vi "Inspector Template [VarMan Spy].vi"() -> ()   [LabVIEW 2021]
doc: "::: CalcExpress Toolkit :::\nCopyright (c) 2000-2026 Konstantin Shifershteyn. All rights reserved."
uses:
  vi.lib/addons/CalcExpress/cetypes.llb/VarMan Variable Context Handle.ctl
  vi.lib/addons/CalcExpress/cemisc.llb/[ce] CE component paths - Kind of Path Enum.ctl
  <vilib>/Utility/miscctls.llb/LVBoundsTypeDef.ctl
panel:
  out "I32B":i32 caption="Bit-keeping conversion" format="%.0x"
  out "I32M":i32 caption="Saturating conversion" format="%.0x"
  out "writerID":u32 caption="writer ID"
  in  "%write":bool
  in  "EnaWrap":bool=TRUE caption="Wrap"
  in  "ShowInt32":bool caption="show I32 and U32"
  out "h_IR":T1(array[cluster]) {"timestamp" format="%<%H:%M:%S%2u\n%d/%m/%Y>T"}
  out "h_any":T2(array[cluster]) {"timestamp" format="%<%H:%M:%S%2u\n%d/%m/%Y>T"}
  out "h_a2str":T3(array[cluster]) {"timestamp" format="%<%H:%M:%S%2u\n%d/%m/%Y>T"}
  out "h_a1str":T4(array[cluster]) {"timestamp" format="%<%H:%M:%S%2u\n%d/%m/%Y>T"}
  out "h_a2cdb":T5(array[cluster]) {"value"."data" format="%.2f"; "timestamp" format="%<%H:%M:%S%2u\n%d/%m/%Y>T"}
  out "h_a1cdb":T6(array[cluster]) {"value"."data" format="%.2f"; "timestamp" format="%<%H:%M:%S%2u\n%d/%m/%Y>T"}
  out "h_cdb":T7(array[cluster]) {"value" format="%.2f"; "timestamp" format="%<%H:%M:%S%2u\n%d/%m/%Y>T"}
  out "h_a2dbl":T8(array[cluster]) {"value"."data" format="%.2f"; "timestamp" format="%<%H:%M:%S%2u\n%d/%m/%Y>T"}
  out "IR":cluster{"Initial index":i32, "Final index":i32} caption="Index Range"
  out "h_a1dbl":T9(array[cluster]) {"value"."data" format="%.2f"; "timestamp" format="%<%H:%M:%S%2u\n%d/%m/%Y>T"}
  in  "bndry":string
  in  "%h_Update":bool caption="update [F2]"
  in  "%h_Auto":bool caption="auto update"
  in  "%h_Reverse":bool=TRUE caption="reversed"
  in  "%h_Show":bool caption="History"
  out "dbl":dbl caption="Value" format="%.2f"
  out "h_str":T2(array[cluster]) caption="Variable History" {"timestamp" format="%<%H:%M:%S%2u\n%d/%m/%Y>T"}
  out "h_dbl":T10(array[cluster]) caption="Variable History" {"value" format="%.2f"; "timestamp" format="%<%H:%M:%S%2u\n%d/%m/%Y>T"}
  in  "alias":string
  out "var type":i32(ring)=10 items=["String"=0, "DBL Number"=1, "Identifier"=2, "1D Array of DBL"=3, "2D Array of DBL"=4, "CDB Number"=5, "1D Array of CDB"=6, "2D Array of CDB"=7, "1D Array of String"=8, "2D Array of String"=9, "Unknown data type"=10, "Index Range"=252]
  in  "var name":string
  out "any":string
  out "a2dbl":dbl[][](array[numeric]) format="%.2f"
  out "a2cdb":cdb[][](array[numeric]) format="%.2f"
  out "cdb":cdb caption="Value" format="%.2f"
  out "a1cdb":cdb[](array[numeric]) format="%.2f"
  out "a1dbl":dbl[](array[numeric]) format="%.2f"
  out "a2str":string[][](array[string])
  out "a1str":string[](array[string])
  in  "Display style":u32(ring) caption="Style" items=["Normal", "'\\' Code", "Password", "Hex dump"]
  out "Update TS":dbl=3131888400.0 format="%<%H:%M:%S%1u>T"
  out "str":string
  in  "Precision":u8=2 caption="prec"
  in  "Format":u8(ring) items=["Floating point", "Scientific", "Engineering", "Binary", "Octal", "Hexadecimal", "Relative time", "Absolute time"]
  in  "%Pause":bool
  out "Context":string
  out "Variable":string
  in  "handle":T11=-1
  # ":"
  # ":"
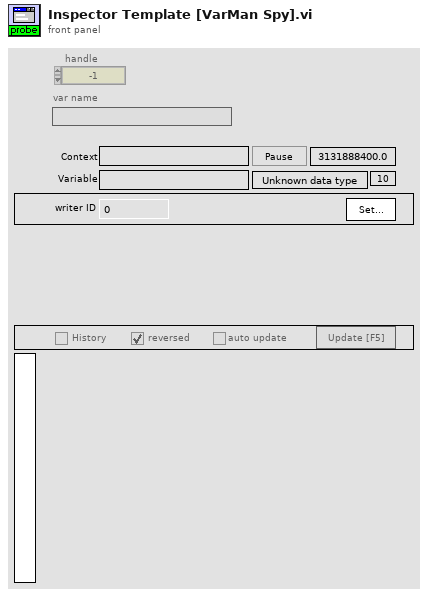
[diagram p1: front panel]
types:
  T1 = cluster{"timestamp":dbl, "IR 2":cluster{"Initial index":i32, "Final index":i32}, "writerID":u32}[]
  T2 = cluster{"timestamp":dbl, "value":string, "writerID":u32}[]
  T3 = cluster{"timestamp":dbl, "value":cluster{"data":string[][]}, "writerID":u32}[]
  T4 = cluster{"timestamp":dbl, "value":cluster{"data":string[]}, "writerID":u32}[]
  T5 = cluster{"timestamp":dbl, "value":cluster{"data":cdb[][]}, "writerID":u32}[]
  T6 = cluster{"timestamp":dbl, "value":cluster{"data":cdb[]}, "writerID":u32}[]
  T7 = cluster{"timestamp":dbl, "value":cdb, "writerID":u32}[]
  T8 = cluster{"timestamp":dbl, "value":cluster{"data":dbl[][]}, "writerID":u32}[]
  T9 = cluster{"timestamp":dbl, "value":cluster{"data":dbl[]}, "writerID":u32}[]
  T10 = cluster{"timestamp":dbl, "value":dbl, "writerID":u32}[]
  T11 = typedef "VarMan Variable Context Handle.ctl" = i32
  T12 = typedef "LVBoundsTypeDef.ctl" = cluster{"Width":u32, "Height":u32}
  T13 = typedef "LVPositionTypeDef.ctl" = cluster{"Left":i32, "Top":i32}
  T14 = typedef "VarMan Variable Data Statistics.ctl" = cluster{"writer ID":u32, "write MS":u32, "write TS":dbl, "write Cnt":u32}
  T15 = cluster{"timestamp":dbl, "value":string, "value":u32}[]
  T16 = cluster{"timestamp":dbl, "value":dbl, "value":u32}[]
  T17 = cluster{"timestamp":dbl, "value":cluster{"data":dbl[]}, "value":u32}[]
  T18 = cluster{"timestamp":dbl, "value":cluster{"data":dbl[][]}, "value":u32}[]
  T19 = cluster{"timestamp":dbl, "value":cdb, "value":u32}[]
  T20 = cluster{"timestamp":dbl, "value":cluster{"data":cdb[]}, "value":u32}[]
  T21 = cluster{"timestamp":dbl, "value":cluster{"data":cdb[][]}, "value":u32}[]
  T22 = cluster{"timestamp":dbl, "value":cluster{"data":string[]}, "value":u32}[]
  T23 = cluster{"timestamp":dbl, "value":cluster{"data":string[][]}, "value":u32}[]
  T24 = cluster{"timestamp":dbl, "Index Range":cluster{"Initial index":i32, "Final index":i32}, "value":u32}[]
  T25 = enum32{"invalid app kind", "Development System", "Run Time System", "Student Edition", "Embedded LabVIEW", "Evaluation", "Custom"}
  T26 = typedef "[ce] CE component paths - Kind of Path Enum.ctl" = enum16{"VIs", "FuncVIs", "Help", "Examples", "Project", "Templates"}
  T27 = enum32{"Invalid", "Standard", "Closed", "Hidden", "Minimized", "Maximized"}
  T28 = typedef "eventvkey.ctl" = enum16{"ASCII", "Enter", "Return", "Shift", "Ctrl", "Alt", "Cmd", "Opt", "Caps", "NumLock", "Clear", "Break", "Up", "Down", "Left", "Right", "Insert", "Delete", "Home", "End", "PageUp", "PageDown", "Escape", "Help", "Pause", "ScrollLock", "F1", "F2", "F3", "F4", "F5", "F6", "F7", "F8", "F9", "F10", "F11", "F12", "F13", "F14", "F15", "F16", "F17", "F18", "F19", "F20", "F21", "F22", "F23", "F24", "Play", "VolumeUp", "VolumeDown", "Mute", "Two Byte Char"}
  T29 = cluster{"Shift":bool, "Ctrl":bool, "Alt":bool, "Cmd":bool, "Opt":bool}
  T30 = typedef "LVRectTypeDef.ctl" = cluster{"Left":i16, "Top":i16, "Right":i16, "Bottom":i16}
  T31 = cluster{"Left":i32, "Top":i32, "Right":i32, "Bottom":i32}
  T32 = cluster{"Value":u8, "Value":u8, "Value":bool, "Value":u32, "Value":bool}
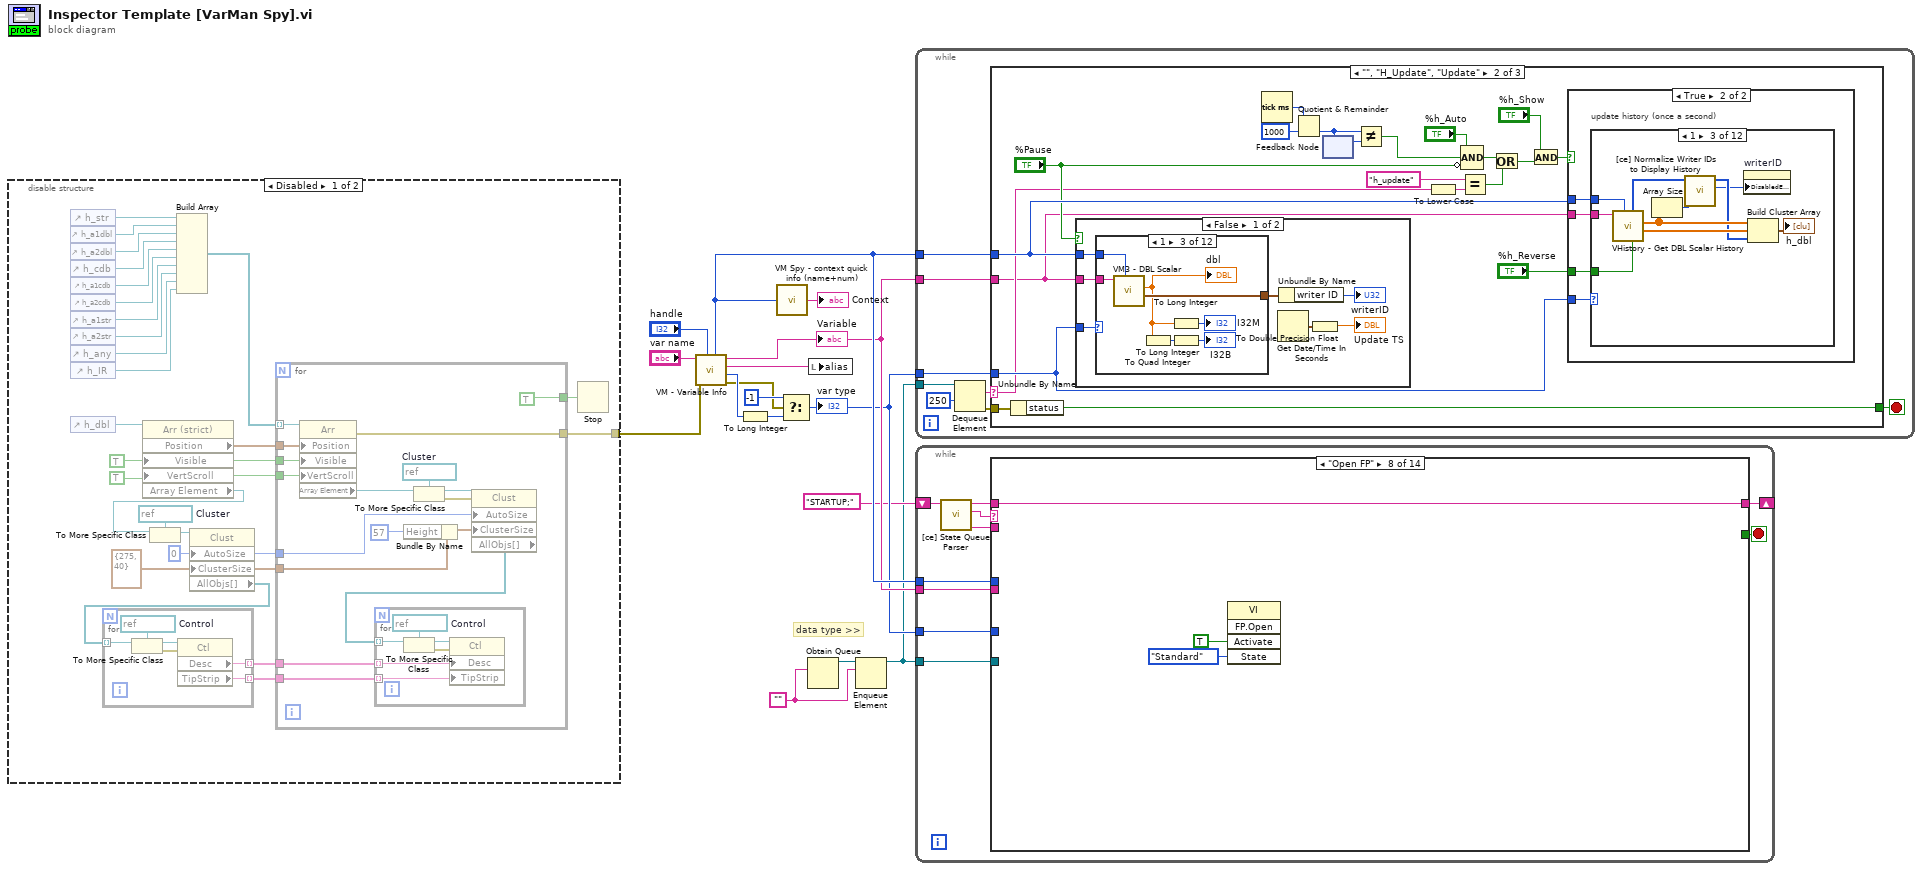
[diagram p0: block diagram]
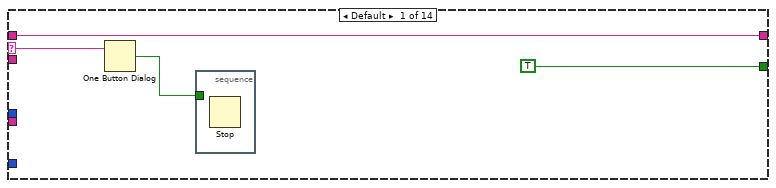
[diagram p3: hidden frame]
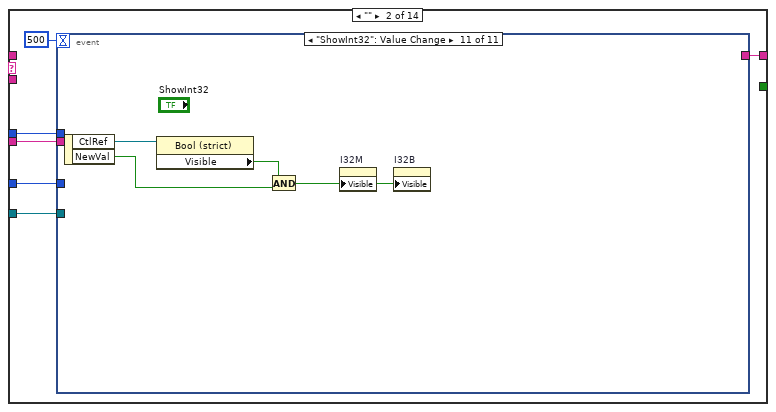
[diagram p4: hidden frame]
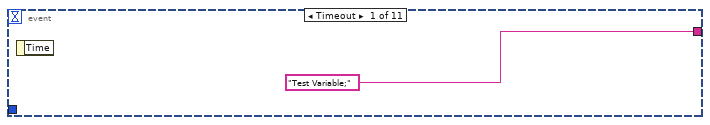
[diagram p5: hidden frame]
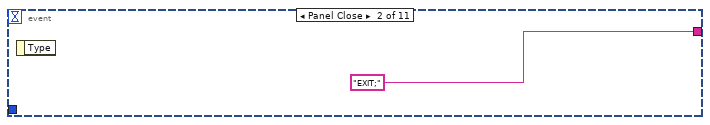
[diagram p6: hidden frame]
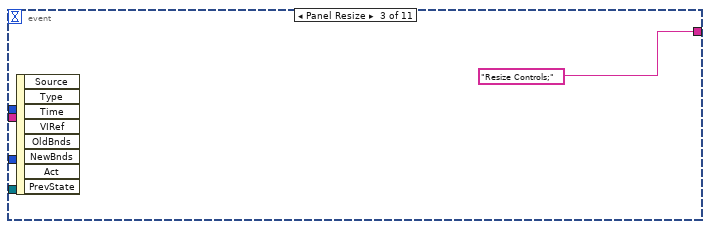
[diagram p7: hidden frame]
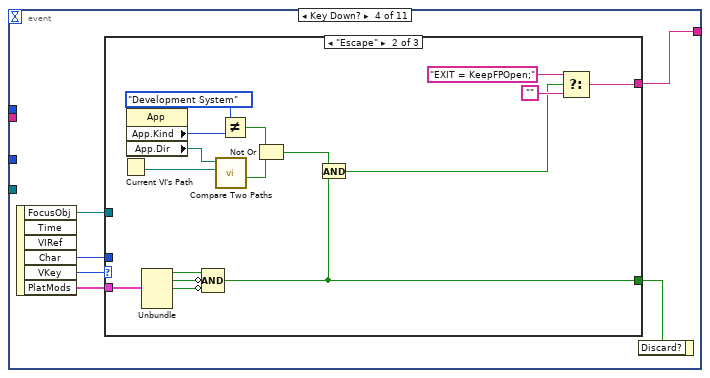
[diagram p8: hidden frame]
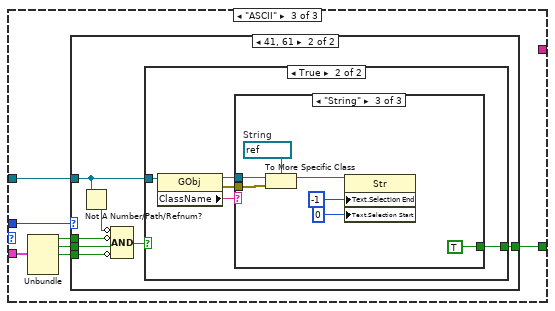
[diagram p10: hidden frame]
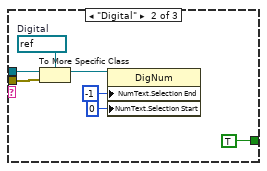
[diagram p14: hidden frame]
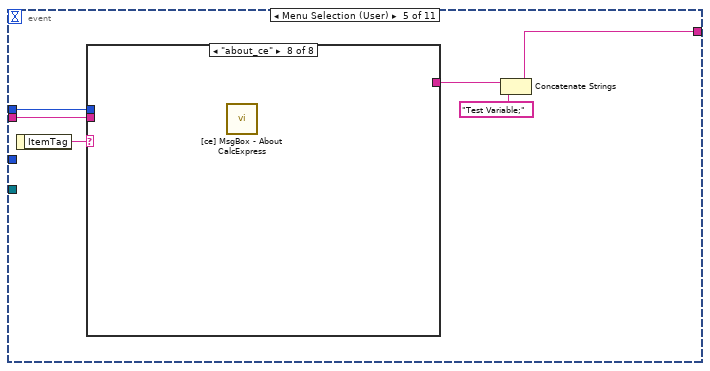
[diagram p15: hidden frame]
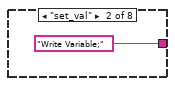
[diagram p17: hidden frame]
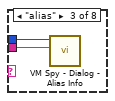
[diagram p18: hidden frame]
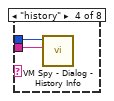
[diagram p19: hidden frame]
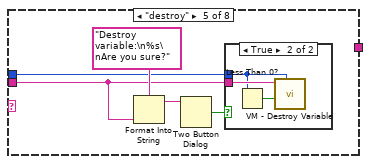
[diagram p20: hidden frame]
diagram:
  w2 = ""
  # "data type >>"
  n1 = disable-structure shown="Disabled" {
    disable-tunnel: [w19 _] -> w1
    frame Disabled {
      w17 = TRUE
      w31 = TRUE ("Visible")
      w27 = T12 {"Width"=275, "Height"=40} ("Cluster Size")
      w26 = u32 0 ("Auto Sizing")
      w23 = refnum<vi> refnum  # Cluster
      n2 = control-ref of="h_str"() -> (w41:refnum<vi>)
      n3 = control-ref of="h_a1dbl"() -> (w40:refnum<vi>)
      n4 = control-ref of="h_a2dbl"() -> (w39:refnum<vi>)
      n5 = control-ref of="h_cdb"() -> (w38:refnum<vi>)
      n6 = control-ref of="h_a1cdb"() -> (w37:refnum<vi>)
      n7 = control-ref of="h_a2cdb"() -> (w36:refnum<vi>)
      n8 = control-ref of="h_a1str"() -> (w35:refnum<vi>)
      n9 = control-ref of="h_a2str"() -> (w34:refnum<vi>)
      n10 = control-ref of="h_any"() -> (w33:refnum<vi>)
      n11 = control-ref of="h_IR"() -> (w32:refnum<vi>)
      n12 = control-ref of="h_dbl"() -> (w21:refnum<vi>)
      n13 = property class="Arr (strict)"(reference=w21, "Visible"=w31, "VertScroll"=w17) -> ("Position"=w22:T13, "Array Element"=w24:refnum<vi>)  [unwired: 1 in, 2 out]
      n14 = To More Specific Class(target class=w23, reference=w24) -> (specific class reference=w25:refnum<vi>)  [unwired: 1 in, 1 out]
      n15 = Build Array(w41, w40, w39, w38, w37, w36, w35, w34, w33, w32) -> (w20:refnum<vi>[])
      n16 = property class="Clust"(reference=w25, "AutoSize"=w26, "ClusterSize"=w27) -> ("AllObjs[]"=w28:refnum<vi>[])  [unwired: 1 in, 2 out]
      n17 = for {
        tunnel: w28 -> [w46] mode=indexing
        tunnel: [w43] -> w29 mode=indexing
        tunnel: [w42] -> w30 mode=indexing
        w47 = refnum<vi> refnum  # Control
        n18 = To More Specific Class(target class=w47, reference=w46) -> (specific class reference=w45:refnum<vi>, error out=w44:errorcluster)  [unwired: 1 in]
        n19 = property class="Ctl"(reference=w45, error in=w44) -> ("Desc"=w43:string, "TipStrip"=w42:string)  [unwired: 2 out]
      }
      n20 = for {
        tunnel: w22 -> [w64]
        tunnel: w20 -> [w63] mode=indexing
        tunnel: w26 -> [w58]
        tunnel: w27 -> [w57]
        tunnel: w29 -> [w53]
        tunnel: w30 -> [w52]
        tunnel: w31 -> [w51]
        tunnel: [w50] -> w19
        tunnel: [TRUE] -> w18
        tunnel: w17 -> [w48]
        w62 = refnum<vi> refnum  # Cluster
        n21 = property class="Arr"(reference=w63, "Position"=w64, "Visible"=w51, "VertScroll"=w48) -> (error out=w50:errorcluster, "Array Element"=w61:refnum<vi>)  [unwired: 1 in, 1 out]
        n22 = Bundle By Name(cluster=w57, "Height"=u32 57) -> (w56:T12)
        n23 = To More Specific Class(target class=w62, reference=w61) -> (specific class reference=w60:refnum<vi>, error out=w59:errorcluster)  [unwired: 1 in]
        n24 = property class="Clust"(reference=w60, error in=w59, "AutoSize"=w58, "ClusterSize"=w56) -> ("AllObjs[]"=w54:refnum<vi>[])  [unwired: 2 out]
        n25 = for {
          tunnel: w54 -> [w69] mode=indexing
          tunnel: w53 -> [w66] mode=indexing
          tunnel: w52 -> [w65] mode=indexing
          w70 = refnum<vi> refnum  # Control
          n26 = To More Specific Class(target class=w70, reference=w69) -> (specific class reference=w68:refnum<vi>, error out=w67:errorcluster)  [unwired: 1 in]
          n27 = property class="Ctl"(reference=w68, error in=w67, "Desc"=w66, "TipStrip"=w65) -> ()  [unwired: 2 out]
        }
      }
      n28 = Stop(stop? (T)=w18) -> ()
    }
    frame Enabled {
    }
  }
  n29 = call "VM - Variable Info.vi"("VC Handle"="handle", "error in"=w1, "name_spec"="var name") -> ("error out"=w5:errorcluster, "var type"=w10:u32, "alias"=w13:string, "var name"=w8:string, "var VC Handle"=w9:T11)  [unwired: 3 in, 1 out]
  "Variable" <- w8
  n30 = To Long Integer(number=w10) -> (32bit integer=w12:i32)
  n31 = call "VM Spy - context quick info (name+num).vi"("handle"=w9) -> ("context info"=→"Context":string)  [unwired: 4 in]
  n32 = Select(t=-1, s=w5, f=w12) -> (s? t:f=w7:i32)
  "var type" <- w7
  n33 = Obtain Queue(element data type=w2) -> (queue out=w4:refnum<queue>)  [unwired: 4 in, 2 out]
  n34 = local write "alias"(w13) -> ()
  n35 = Enqueue Element(queue=w4, element=w2) -> (queue out=w3:refnum<queue>)  [unwired: 2 in, 2 out]
  n36 = while {
    tunnel: w8 -> [w78]
    tunnel: w9 -> [w76]
    tunnel: w7 -> [w77]
    tunnel: w3 -> [w75]
    stop <- w72 stop-if-true
    n37 = Dequeue Element(queue=w75, timeout in ms (-1)=250) -> (element=w74:string, error out=w71:errorcluster)  [unwired: 1 in, 2 out]
    n38 = case shown="\"\", \"H_Update\", \"Update\"" w74 {
      selector: w74 -> [_ w84 _]
      tunnel: w78 -> [_ w80 _]
      tunnel: w77 -> [_ w100 _]
      tunnel: w76 -> [_ w99 _]
      tunnel: [TRUE w86 w278] -> w72
      tunnel: w71 -> [_ w87 w279]
      frame "EXIT" {
      }
      frame "", "H_Update", "Update" {
        n39 = Unbundle By Name(w87) -> ("status"=w86:bool)
        n40 = case shown="False" "%Pause" {
          tunnel: w99 -> [w224 _]
          tunnel: w80 -> [w222 _]
          tunnel: w100 -> [w221 _]
          frame False {
            n41 = case shown="1" w221 {
              selector: w221 -> [_ _ _ _ _ _ _ _ _ _ w270 w276]
              tunnel: w222 -> [w227 w231 w238 w242 w246 w250 w254 w258 w262 w266 w271 w277]
              tunnel: w224 -> [w226 w229 w237 w240 w244 w248 w252 w256 w260 w264 w268 w273]
              tunnel: [w225 w228 w236 w239 w243 w247 w251 w255 w259 w263 w267 w272] -> w219
              frame -1, 2 {
                n42 = call "VM3 - Variable Data Info.vi"("VC Handle"=w226, "name_spec"=w227) -> ("stats"=w225:T14)  [unwired: 4 in, 5 out]
              }
              frame 0 {
                n43 = call "VM3 - String.vi"("VC Handle"=w229, "name_spec"=w231) -> ("stats"=w228:T14, "value out"=→"str":string)  [unwired: 6 in, 2 out]
              }
              frame 1 {
                n44 = call "VM3 - DBL Scalar.vi"("VC Handle"=w237, "name_spec"=w238) -> ("stats"=w236:T14, "value out"=w234:dbl)  [unwired: 6 in, 2 out]
                "dbl" <- w234
                n45 = To Quad Integer(1:w234) -> (0:w235:i64)
                n46 = To Long Integer(number=w234) -> (32bit integer=→"I32M":i32)
                n47 = To Long Integer(number=w235) -> (32bit integer=→"I32B":i32)
              }
              frame 3 {
                n48 = call "VM3 - 1D Array of DBL.vi"("VC Handle"=w240, "name_spec"=w242) -> ("stats"=w239:T14, "value out"=→"a1dbl":dbl[])  [unwired: 6 in, 2 out]
              }
              frame 4 {
                n49 = call "VM3 - 2D Array of DBL.vi"("VC Handle"=w244, "name_spec"=w246) -> ("stats"=w243:T14, "value out"=→"a2dbl":dbl[][])  [unwired: 6 in, 2 out]
              }
              frame 5 {
                n50 = call "VM3 - CDB Scalar.vi"("VC Handle"=w248, "name_spec"=w250) -> ("stats"=w247:T14, "value out"=→"cdb":cdb)  [unwired: 6 in, 2 out]
              }
              frame 6 {
                n51 = call "VM3 - 1D Array of CDB.vi"("VC Handle"=w252, "name_spec"=w254) -> ("stats"=w251:T14, "value out"=→"a1cdb":cdb[])  [unwired: 6 in, 2 out]
              }
              frame 7 {
                n52 = call "VM3 - 2D Array of CDB.vi"("VC Handle"=w256, "name_spec"=w258) -> ("stats"=w255:T14, "value out"=→"a2cdb":cdb[][])  [unwired: 6 in, 2 out]
              }
              frame 8 {
                n53 = call "VM3 - 1D Array of Strings.vi"("VC Handle"=w260, "name_spec"=w262) -> ("stats"=w259:T14, "value out"=→"a1str":string[])  [unwired: 6 in, 2 out]
              }
              frame 9 {
                n54 = call "VM3 - 2D Array of Strings.vi"("VC Handle"=w264, "name_spec"=w266) -> ("stats"=w263:T14, "value out"=→"a2str":string[][])  [unwired: 6 in, 2 out]
              }
              frame 10, Default {
                n55 = call "VM3 - Arbitrary Data.vi"("var type in"=w270, "VC Handle"=w268, "name_spec"=w271) -> ("stats"=w267:T14, "flattened value out"=→"any":string)  [unwired: 4 in, 3 out]
              }
              frame 252 {
                n56 = call "VM3 - Arbitrary Data.vi"("var type in"=w276, "VC Handle"=w273, "name_spec"=w277) -> ("stats"=w272:T14, "flattened value out"=w275:string)  [unwired: 4 in, 3 out]
                n57 = call "[ce] Index Range from Flattened String.vi"("Flattened string"=w275) -> ("Index Range"=→"IR":cluster{"Initial index":i32, "Final index":i32})  [unwired: 10 in]
              }
            }
            n58 = Get Date/Time In Seconds() -> (seconds since 1Jan1904=w220:timestamp)
            n59 = Unbundle By Name(w219) -> ("writer ID"=→"writerID":u32)
            n60 = To Double Precision Float(number=w220) -> (double precision float=→"Update TS":dbl)
          }
          frame True {
          }
        }
        n61 = Tick Count (ms)() -> (millisecond timer value=w98:u32)
        n62 = Quotient & Remainder(x=w98, y=u32 1000) -> (floor(x/y)=w89:u32)  [unwired: 1 out]
        n63 = feedback-in #1(w89) -> ()
        n64 = feedback #1() -> (w90:u32)  [unwired: 1 in]
        n65 = Not Equal?(x=w89, y=w90) -> (x != y?=w88:bool)
        n66 = To Lower Case(string=w84) -> (all lower case string=w81:string)
        n67 = Equal?(x="h_update", y=w81) -> (x = y?=w82:bool)
        n68 = Compound Arithmetic op=AND("%h_Auto", w88, invert "%Pause") -> (w85:bool)
        n69 = Or(x=w85, y=w82) -> (x .or. y?=w92:bool)
        n70 = And(x="%h_Show", y=w92) -> (x .and. y?=w97:bool)
        n71 = case shown="True" w97 {
          tunnel: w80 -> [_ w103]
          tunnel: w100 -> [_ w104]
          tunnel: w99 -> [_ w102]
          tunnel: "%h_Reverse" -> [_ w101]
          frame False {
          }
          frame True {
            # "update history (once a second)"
            n72 = case shown="1" w104 {
              tunnel: w103 -> [_ w114 w124 w134 w144 w154 w164 w174 w184 w194 w204 w215]
              tunnel: w102 -> [_ w113 w123 w133 w143 w153 w163 w173 w183 w193 w203 w214]
              tunnel: w101 -> [_ w110 w120 w130 w141 w151 w161 w171 w181 w191 w201 w213]
              frame -1, 2 {
              }
              frame 0 {
                n73 = call "VHistory - Get STR History.vi"("reverse order (T)"=w110, "VC Handle"=w113, "name_spec"=w114) -> ("history"=w112:string[], "time stamps"=w108:dbl[], "writer IDs"=w107:u32[])  [unwired: 4 in, 2 out]
                n74 = Array Size(array=w108) -> (size(s)=w109:i32)
                n75 = call "[ce] Normalize Writer IDs to Display History.vi"("size"=w109, "writer IDs in"=w107) -> ("disable"=w105:u8, "writer IDs"=w106:u32[])  [unwired: 8 in]
                n76 = Build Cluster Array(w108, w112, w106) -> (→"h_str":T15)
                n77 = property on="writerID" class="DigNum (strict)"("DisabledEnum"=w105) -> ()  [unwired: 2 in, 2 out]
              }
              frame 1 {
                n78 = call "VHistory - Get DBL Scalar History.vi"("reverse order (T)"=w120, "VC Handle"=w123, "name_spec"=w124) -> ("history"=w122:dbl[], "time stamps"=w118:dbl[], "writer IDs"=w117:u32[])  [unwired: 4 in, 2 out]
                n79 = Array Size(array=w118) -> (size(s)=w119:i32)
                n80 = call "[ce] Normalize Writer IDs to Display History.vi"("size"=w119, "writer IDs in"=w117) -> ("disable"=w115:u8, "writer IDs"=w116:u32[])  [unwired: 8 in]
                n81 = property on="writerID" class="DigNum (strict)"("DisabledEnum"=w115) -> ()  [unwired: 2 in, 2 out]
                n82 = Build Cluster Array(w118, w122, w116) -> (→"h_dbl":T16)
              }
              frame 3 {
                n83 = call "VHistory - Get 1D Array of DBL History.vi"("reverse order (T)"=w130, "VC Handle"=w133, "name_spec"=w134) -> ("history"=w132:cluster{"data":dbl[]}[], "time stamps"=w128:dbl[], "writer IDs"=w127:u32[])  [unwired: 4 in, 2 out]
                n84 = Array Size(array=w128) -> (size(s)=w129:i32)
                n85 = call "[ce] Normalize Writer IDs to Display History.vi"("size"=w129, "writer IDs in"=w127) -> ("disable"=w125:u8, "writer IDs"=w126:u32[])  [unwired: 8 in]
                n86 = property on="writerID" class="DigNum (strict)"("DisabledEnum"=w125) -> ()  [unwired: 2 in, 2 out]
                n87 = Build Cluster Array(w128, w132, w126) -> (→"h_a1dbl":T17)
              }
              frame 4 {
                n88 = call "VHistory - Get 2D Array of DBL History.vi"("reverse order (T)"=w141, "VC Handle"=w143, "name_spec"=w144) -> ("history"=w142:cluster{"data":dbl[][]}[], "time stamps"=w138:dbl[], "writer IDs"=w137:u32[])  [unwired: 4 in, 2 out]
                n89 = Array Size(array=w138) -> (size(s)=w139:i32)
                n90 = call "[ce] Normalize Writer IDs to Display History.vi"("size"=w139, "writer IDs in"=w137) -> ("disable"=w135:u8, "writer IDs"=w136:u32[])  [unwired: 8 in]
                n91 = property on="writerID" class="DigNum (strict)"("DisabledEnum"=w135) -> ()  [unwired: 2 in, 2 out]
                n92 = Build Cluster Array(w138, w142, w136) -> (→"h_a2dbl":T18)
              }
              frame 5 {
                n93 = call "VHistory - Get CDB Scalar History.vi"("reverse order (T)"=w151, "VC Handle"=w153, "name_spec"=w154) -> ("history"=w152:cdb[], "time stamps"=w148:dbl[], "writer IDs"=w147:u32[])  [unwired: 4 in, 2 out]
                n94 = Array Size(array=w148) -> (size(s)=w149:i32)
                n95 = call "[ce] Normalize Writer IDs to Display History.vi"("size"=w149, "writer IDs in"=w147) -> ("disable"=w145:u8, "writer IDs"=w146:u32[])  [unwired: 8 in]
                n96 = property on="writerID" class="DigNum (strict)"("DisabledEnum"=w145) -> ()  [unwired: 2 in, 2 out]
                n97 = Build Cluster Array(w148, w152, w146) -> (→"h_cdb":T19)
              }
              frame 6 {
                n98 = call "VHistory - Get 1D Array of CDB History.vi"("reverse order (T)"=w161, "VC Handle"=w163, "name_spec"=w164) -> ("history"=w162:cluster{"data":cdb[]}[], "time stamps"=w158:dbl[], "writer IDs"=w157:u32[])  [unwired: 4 in, 2 out]
                n99 = Array Size(array=w158) -> (size(s)=w159:i32)
                n100 = call "[ce] Normalize Writer IDs to Display History.vi"("size"=w159, "writer IDs in"=w157) -> ("disable"=w155:u8, "writer IDs"=w156:u32[])  [unwired: 8 in]
                n101 = property on="writerID" class="DigNum (strict)"("DisabledEnum"=w155) -> ()  [unwired: 2 in, 2 out]
                n102 = Build Cluster Array(w158, w162, w156) -> (→"h_a1cdb":T20)
              }
              frame 7 {
                n103 = call "VHistory - Get 2D Array of CDB History.vi"("reverse order (T)"=w171, "VC Handle"=w173, "name_spec"=w174) -> ("history"=w172:cluster{"data":cdb[][]}[], "time stamps"=w167:dbl[], "writer IDs"=w168:u32[])  [unwired: 4 in, 2 out]
                n104 = Array Size(array=w167) -> (size(s)=w169:i32)
                n105 = call "[ce] Normalize Writer IDs to Display History.vi"("size"=w169, "writer IDs in"=w168) -> ("disable"=w165:u8, "writer IDs"=w166:u32[])  [unwired: 8 in]
                n106 = property on="writerID" class="DigNum (strict)"("DisabledEnum"=w165) -> ()  [unwired: 2 in, 2 out]
                n107 = Build Cluster Array(w167, w172, w166) -> (→"h_a2cdb":T21)
              }
              frame 8 {
                n108 = call "VHistory - Get 1D Array of STR History.vi"("reverse order (T)"=w181, "VC Handle"=w183, "name_spec"=w184) -> ("history"=w182:cluster{"data":string[]}[], "time stamps"=w178:dbl[], "writer IDs"=w177:u32[])  [unwired: 4 in, 2 out]
                n109 = Array Size(array=w178) -> (size(s)=w179:i32)
                n110 = call "[ce] Normalize Writer IDs to Display History.vi"("size"=w179, "writer IDs in"=w177) -> ("disable"=w175:u8, "writer IDs"=w176:u32[])  [unwired: 8 in]
                n111 = property on="writerID" class="DigNum (strict)"("DisabledEnum"=w175) -> ()  [unwired: 2 in, 2 out]
                n112 = Build Cluster Array(w178, w182, w176) -> (→"h_a1str":T22)
              }
              frame 9 {
                n113 = call "VHistory - Get 2D Array of STR History.vi"("reverse order (T)"=w191, "VC Handle"=w193, "name_spec"=w194) -> ("history"=w192:cluster{"data":string[][]}[], "time stamps"=w188:dbl[], "writer IDs"=w187:u32[])  [unwired: 4 in, 2 out]
                n114 = Array Size(array=w188) -> (size(s)=w189:i32)
                n115 = call "[ce] Normalize Writer IDs to Display History.vi"("size"=w189, "writer IDs in"=w187) -> ("disable"=w185:u8, "writer IDs"=w186:u32[])  [unwired: 8 in]
                n116 = property on="writerID" class="DigNum (strict)"("DisabledEnum"=w185) -> ()  [unwired: 2 in, 2 out]
                n117 = Build Cluster Array(w188, w192, w186) -> (→"h_a2str":T23)
              }
              frame 10, Default {
                n118 = call "VHistory - Get Arbitrary Variable History.vi"("reverse order (T)"=w201, "VC Handle"=w203, "name_spec"=w204) -> ("history"=w202:string[], "time stamps"=w198:dbl[], "writer IDs"=w197:u32[])  [unwired: 4 in, 2 out]
                n119 = Array Size(array=w198) -> (size(s)=w199:i32)
                n120 = call "[ce] Normalize Writer IDs to Display History.vi"("size"=w199, "writer IDs in"=w197) -> ("disable"=w195:u8, "writer IDs"=w196:u32[])  [unwired: 8 in]
                n121 = property on="writerID" class="DigNum (strict)"("DisabledEnum"=w195) -> ()  [unwired: 2 in, 2 out]
                n122 = Build Cluster Array(w198, w202, w196) -> (→"h_any":T15)
              }
              frame 252 {
                n123 = call "VHistory - Get Arbitrary Variable History.vi"("reverse order (T)"=w213, "VC Handle"=w214, "name_spec"=w215) -> ("history"=w212:string[], "time stamps"=w208:dbl[], "writer IDs"=w207:u32[])  [unwired: 4 in, 2 out]
                n124 = Array Size(array=w208) -> (size(s)=w209:i32)
                n125 = for {
                  tunnel: w212 -> [w217] mode=indexing
                  tunnel: [w216] -> w211 mode=indexing
                  n126 = call "[ce] Index Range from Flattened String.vi"("Flattened string"=w217) -> ("Index Range"=w216:cluster{"Initial index":i32, "Final index":i32})  [unwired: 10 in]
                }
                n127 = call "[ce] Normalize Writer IDs to Display History.vi"("size"=w209, "writer IDs in"=w207) -> ("disable"=w205:u8, "writer IDs"=w206:u32[])  [unwired: 8 in]
                n128 = property on="writerID" class="DigNum (strict)"("DisabledEnum"=w205) -> ()  [unwired: 2 in, 2 out]
                n129 = Build Cluster Array(w208, w211, w206) -> (→"h_IR":T24)
              }
            }
          }
        }
      }
      frame Default {
        n130 = Unbundle By Name(w279) -> ("status"=w278:bool)
      }
    }
  }
  n131 = while {
    tunnel: w9 -> [w289]
    tunnel: w8 -> [w288]
    tunnel: w7 -> [w287]
    shift-right: [w283] -> _
    shift-left: "STARTUP;" -> [w286]
    tunnel: w3 -> [w281]
    stop <- w284 stop-if-true
    n132 = call "[ce] State Queue Parser.vi"("input queue"=w286) -> ("state parameters"=w280:string, "state"=w285:string, "remained queue"=w282:string)  [unwired: 6 in]
    n133 = case shown="\"Open FP\"" w285 {
      selector: w285 -> [w292 _ _ _ _ _ _ _ _ _ _ _ _ _]
      tunnel: w289 -> [_ w299 _ _ _ _ _ _ _ _ _ _ w627 w646]
      tunnel: w288 -> [_ w298 _ _ _ _ _ _ _ _ _ _ w626 w645]
      tunnel: w287 -> [_ w297 _ w430 _ _ _ _ _ w535 _ _ _ _]
      tunnel: [TRUE _ _ _ _ TRUE _ _ _ _ _ _ _ _] -> w284
      tunnel: [w290 w295 w425 w435 w506 w510 w511 w514 w519 w541 w614 w615 w622 w653] -> w283
      tunnel: w282 -> [w290 _ w426 w435 w507 w510 w511 w514 w533 w541 w614 w615 w616 w653]
      tunnel: w281 -> [_ w294 _ _ w504 w508 _ _ _ _ _ _ _ _]
      tunnel: w280 -> [_ _ _ _ w502 _ _ _ _ _ _ _ _ _]
      frame Default {
        n134 = One Button Dialog(message=w292) -> (true=w291:bool)  [unwired: 1 in]
        n135 = stacked-sequence {
          tunnel: w291 -> [_]
          frame #0 {
            n136 = Stop() -> ()  [unwired: 1 in]
          }
        }
      }
      frame "" {
        n137 = event shown="[10] \"ShowInt32\": Value Change" {
          selector: _ -> [_ _ _ _ _ _ _ _ _ _ _]
          dyn-events: _ -> [_ _ _ _ _ _ _ _ _ _ _]
          timeout: 500 -> [_ _ _ _ _ _ _ _ _ _ _]
          tunnel: w299 -> [_ _ _ _ w362 _ _ _ _ _ _]
          tunnel: w298 -> [_ _ _ _ w361 _ _ _ _ _ _]
          tunnel: w297 -> [_ _ _ _ _ _ _ _ _ w397 _]
          tunnel: ["Test Variable;" "EXIT;" "Resize Controls;" w305 w359 "Write Variable;" "Set Window Size;\nControl Appearance;" _ _ _ _] -> w295
          tunnel: w294 -> [_ _ _ _ _ _ w385 w389 w392 _ _]
          event Timeout {
            n138 = event-data() -> ()  [unwired: 1 in, 1 out]
          }
          event Panel Close {
            n139 = event-data() -> ()  [unwired: 1 in, 1 out]
          }
          event Panel Resize {
            n140 = event-data() -> ()  [unwired: 1 in, 8 out]
          }
          event Key Down? {
            n141 = event-data() -> ("FocusObj"=w303:refnum<vi>, "Char"=w304:i16, "VKey"=w308:T28, "PlatMods"=w307:T29)  [unwired: 1 in, 2 out]
            n142 = case shown="\"Escape\"" w308 {
              tunnel: w307 -> [_ w324 w331]
              tunnel: [_ w310 w325] -> w306
              tunnel: [_ w318 _] -> w305
              tunnel: w304 -> [_ _ w327]
              tunnel: w303 -> [_ _ w326]
              frame Default {
              }
              frame "Escape" {
                n143 = Current VI's Path() -> (path=w317:path)
                n144 = property class="App"() -> ("App.Kind"=w315:T25, "App.Dir"=w316:path)  [unwired: 2 in, 2 out]
                n145 = Unbundle(w324) -> ("Shift"=w323:bool, "Ctrl"=w322:bool, "Alt"=w321:bool)  [unwired: 2 out]
                n146 = Compound Arithmetic op=AND(w323, invert w322, invert w321) -> (w310:bool)
                n147 = call <vilib>:"Compare Two Paths.vi"("Path 2"=w317, "Path 1"=w316) -> ("Path 2 Relative to Path 1?"=w313:bool)  [unwired: 6 in, 3 out]
                n148 = Not Equal?(x=T25."Development System", y=w315) -> (x != y?=w314:bool)
                n149 = Not Or(1:w313, 2:w314) -> (0:w312:bool)
                n150 = And(x=w312, y=w310) -> (x .and. y?=w309:bool)
                n151 = Select(t="EXIT = KeepFPOpen;", s=w309, f="") -> (s? t:f=w318:string)
              }
              frame "ASCII" {
                n152 = Unbundle(w331) -> ("Shift"=w330:bool, "Ctrl"=w329:bool, "Alt"=w328:bool)  [unwired: 2 out]
                n153 = case shown="41, 61" w327 {
                  tunnel: w330 -> [_ w338]
                  tunnel: w329 -> [_ w337]
                  tunnel: w328 -> [_ w336]
                  tunnel: w326 -> [_ w333]
                  tunnel: [_ w332] -> w325
                  frame Default {
                  }
                  frame 65, 97 {
                    n154 = Not A Number/Path/Refnum?(number/path/refnum=w333) -> (NaN/Path/Refnum?=w335:bool)
                    n155 = Compound Arithmetic op=AND(invert w335, invert w338, w337, invert w336) -> (w334:bool)
                    n156 = case shown="True" w334 {
                      tunnel: w333 -> [_ w343]
                      tunnel: [_ w341] -> w332
                      frame False {
                      }
                      frame True {
                        n157 = property class="GObj"(reference=w343) -> (reference out=w340:refnum<vi>, error out=w339:errorcluster, "ClassName"=w342:string)  [unwired: 1 in]
                        n158 = case shown="\"String\"" w342 {
                          tunnel: [_ TRUE TRUE] -> w341
                          tunnel: w340 -> [_ w348 w355]
                          tunnel: w339 -> [_ w347 w354]
                          frame Default {
                          }
                          frame "Digital" {
                            w349 = refnum<vi> refnum  # Digital
                            n159 = To More Specific Class(target class=w349, reference=w348, error in=w347) -> (specific class reference=w346:refnum<vi>)  [unwired: 1 out]
                            n160 = property class="DigNum"(reference=w346, "NumText.Selection End"=-1 ("Numeric Text.Selection:End"), "NumText.Selection Start"=u32 0 ("Numeric Text.Selection:Start")) -> ()  [unwired: 1 in, 2 out]
                          }
                          frame "String" {
                            w356 = refnum<vi> refnum  # String
                            n161 = To More Specific Class(target class=w356, reference=w355, error in=w354) -> (specific class reference=w353:refnum<vi>)  [unwired: 1 out]
                            n162 = property class="Str"(reference=w353, "Text.Selection End"=-1 ("Numeric Text.Selection:End"), "Text.Selection Start"=u32 0 ("Numeric Text.Selection:Start")) -> ()  [unwired: 1 in, 2 out]
                          }
                        }
                      }
                    }
                  }
                }
              }
            }
            n163 = event-data("Discard?"=w306) -> ()  [unwired: 1 in, 1 out]
          }
          event Menu Selection (User) {
            n164 = event-data() -> ("ItemTag"=w363:string)  [unwired: 1 in]
            n165 = case shown="\"about_ce\"" w363 {
              tunnel: w362 -> [_ _ w366 w368 w369 _ _ _]
              tunnel: w361 -> [_ _ w365 w367 w370 _ _ _]
              tunnel: [_ "Write Variable;" _ _ _ "EXIT;" _ _] -> w360
              frame "", Default {
              }
              frame "set_val" {
              }
              frame "alias" {
                n166 = call "VM Spy - Dialog - Alias Info.vi"("var name"=w365, "vc handle"=w366) -> ()  [unwired: 9 in, 1 out]
              }
              frame "history" {
                n167 = call "VM Spy - Dialog - History Info.vi"("var name"=w367, "vc handle"=w368) -> ()  [unwired: 7 in, 1 out]
              }
              frame "destroy" {
                n168 = Format Into String(format string="Destroy variable:\n%s\nAre you sure?", w370) -> (resulting string=w372:string)  [unwired: 2 in, 1 out]
                n169 = Two Button Dialog(message=w372) -> (T button?=w371:bool)  [unwired: 2 in]
                n170 = case shown="True" w371 {
                  tunnel: w370 -> [_ w376]
                  tunnel: w369 -> [_ w374]
                  frame False {
                  }
                  frame True {
                    n171 = Less Than 0?(x=w374) -> (x < 0?=w375:bool)
                    n172 = call "VM - Destroy Variable.vi"("VC Handle"=w374, "global ? (F)"=w375, "name_spec"=w376) -> ()  [unwired: 5 in, 4 out]
                  }
                }
              }
              frame "close" {
              }
              frame "help_vi" {
                n173 = call "[ce] CE component paths.vi"("kind of path"=[ce]_CE_component_paths_-_Kind_of_Path_Enum."Help", "append path"="CEToolkit.chm") -> ("path out"=w381:path)
                n174 = Control Online Help(2:w381, 3:"varman_spy.html#vmspy_inspector" ("String to search for"), 4:enum16{"Contents", "Key", "Close"}."Key" ("Operation")) -> ()  [unwired: 1 in, 1 out]
              }
              frame "about_ce" {
                n175 = call "[ce] MsgBox - About CalcExpress.vi"() -> ()  [unwired: 11 in, 1 out]
              }
            }
            n176 = Concatenate Strings(w360, "Test Variable;") -> (w359:string)
          }
          event "%write": Value Change {
            n177 = event-data() -> ()  [unwired: 1 in, 6 out]
          }
          event "%h_Show": Value Change {
            n178 = event-data() -> ("NewVal"=w384:bool)  [unwired: 1 in]
            n179 = case shown="True" w384 {
              tunnel: w385 -> [_ w387]
              frame False {
              }
              frame True {
                n180 = Enqueue Element(queue=w387, element="H_Update") -> ()  [unwired: 2 in, 3 out]
              }
            }
          }
          event "%h_Reverse": Value Change {
            n181 = event-data() -> ()  [unwired: 1 in, 1 out]
            n182 = Enqueue Element(queue=w389, element="H_Update") -> ()  [unwired: 2 in, 3 out]
          }
          event "%h_Update": Value Change {
            n183 = event-data() -> ()  [unwired: 1 in, 1 out]
            n184 = Enqueue Element(queue=w392, element="H_Update") -> ()  [unwired: 2 in, 3 out]
          }
          event "Format", "Precision", "Display style", "EnaWrap": Value Change {
            n185 = event-data() -> ()  [unwired: 1 in, 3 out]
            n186 = case shown="0" w397 {
              tunnel: "Format" -> [_ _ w402 w404 w406 w408 w410 w412 _ _ _ _]
              tunnel: "Precision" -> [_ _ w401 w403 w405 w407 w409 w411 _ _ _ _]
              tunnel: "Display style" -> [_ w400 _ _ _ _ _ _ w413 w414 w415 _]
              tunnel: "EnaWrap" -> [_ w398 _ _ _ _ _ _ _ _ _ _]
              frame -1, 2 {
              }
              frame 0 {
                n187 = Not(x=w398) -> (.not. x?=w399:bool)
                n188 = property on="str" class="Str"("Display Style"=w400, "WrappingEnabled"=w398, "HScrollVis"=w399) -> ()  [unwired: 2 in, 2 out]
                n189 = property on="value" class="Str"("Display Style"=w400) -> ()  [unwired: 2 in, 2 out]
              }
              frame 1 {
                n190 = property on="dbl" class="DigNum (strict)"("Display Format:Format"=w402, "Display Format:Precision"=w401) -> ()  [unwired: 2 in, 2 out]
                n191 = property on="value" class="DigNum (strict)"("Display Format:Format"=w402, "Display Format:Precision"=w401) -> ()  [unwired: 2 in, 2 out]
              }
              frame 3 {
                n192 = property on="dbl" class="DigNum (strict)"("Display Format:Format"=w404, "Display Format:Precision"=w403) -> ()  [unwired: 2 in, 2 out]
                n193 = property class="DigNum (strict)"("Display Format:Format"=w404, "Display Format:Precision"=w403) -> ()  [unwired: 2 in, 2 out]
              }
              frame 4 {
                n194 = property on="dbl" class="DigNum (strict)"("Display Format:Format"=w406, "Display Format:Precision"=w405) -> ()  [unwired: 2 in, 2 out]
                n195 = property class="DigNum (strict)"("Display Format:Format"=w406, "Display Format:Precision"=w405) -> ()  [unwired: 2 in, 2 out]
              }
              frame 5 {
                n196 = property on="cdb" class="DigNum (strict)"("Display Format:Format"=w408, "Display Format:Precision"=w407) -> ()  [unwired: 2 in, 2 out]
                n197 = property on="value" class="DigNum (strict)"("Display Format:Format"=w408, "Display Format:Precision"=w407) -> ()  [unwired: 2 in, 2 out]
              }
              frame 6 {
                n198 = property on="dbl" class="DigNum (strict)"("Display Format:Format"=w410, "Display Format:Precision"=w409) -> ()  [unwired: 2 in, 2 out]
                n199 = property class="DigNum (strict)"("Display Format:Format"=w410, "Display Format:Precision"=w409) -> ()  [unwired: 2 in, 2 out]
              }
              frame 7 {
                n200 = property on="dbl" class="DigNum (strict)"("Display Format:Format"=w412, "Display Format:Precision"=w411) -> ()  [unwired: 2 in, 2 out]
                n201 = property class="DigNum (strict)"("Display Format:Format"=w412, "Display Format:Precision"=w411) -> ()  [unwired: 2 in, 2 out]
              }
              frame 8 {
                n202 = property class="Str"("Display Style"=w413) -> ()  [unwired: 2 in, 2 out]
                n203 = property class="Str"("Display Style"=w413) -> ()  [unwired: 2 in, 2 out]
              }
              frame 9 {
                n204 = property class="Str"("Display Style"=w414) -> ()  [unwired: 2 in, 2 out]
                n205 = property class="Str"("Display Style"=w414) -> ()  [unwired: 2 in, 2 out]
              }
              frame 10, Default {
                n206 = property on="any" class="Str"("Display Style"=w415) -> ()  [unwired: 2 in, 2 out]
                n207 = property on="value" class="Str"("Display Style"=w415) -> ()  [unwired: 2 in, 2 out]
              }
              frame 252 {
              }
            }
          }
          event "ShowInt32": Value Change {
            n208 = event-data() -> ("CtlRef"=w419:refnum<vi>, "NewVal"=w417:bool)  [unwired: 1 in]
            n209 = property on="Property Node" class="Bool (strict)"(reference=w419) -> ("Visible"=w418:bool)  [unwired: 1 in, 2 out]
            n210 = And(x=w418, y=w417) -> (x .and. y?=w416:bool)
            n211 = property on="I32M" class="DigNum (strict)"("Visible"=w416) -> ()  [unwired: 2 in, 2 out]
            n212 = property on="I32B" class="DigNum (strict)"("Visible"=w416) -> ()  [unwired: 2 in, 2 out]
          }
        }
      }
      frame "STARTUP" {
        n213 = local write "%h_Show"(FALSE ("History")) -> ()
        n214 = local write "%h_Reverse"(TRUE ("reversed")) -> ()
        n215 = Current VI's Menubar() -> (w421:refnum<k9>)
        n216 = call "[ce] Create menu at runtime.vi"("menu descriptor"="> _Spy : spy\n  _Set Value... : set_val : key=S\n  ---\n  _Alias... : alias\n  _History... : history\n  _Destroy... : destroy\n  ---\n  _Close : close : key=.\n<\n> Windows : APP_WINDOWS\n  Open Windows * : APP_OPEN_WINDOWS\n<\n> _Help : APP_HELP\n   Help for Variable Inspector : help_vi\n   ---\n   About CalcExpress.. : about_ce\n<\n", "menu"=w421) -> ()  [unwired: 8 in, 2 out]
        n217 = Concatenate Strings("INIT;\n\nSet Window Size;\nControl Appearance;\n\nTest Variable;\n\nOpen FP;" ("string"), w426) -> (w425:string)
      }
      frame "INIT" {
        w427 = 2  # Identifier
        w432 = FALSE
        n218 = Equal?(x=w430, y=w427) -> (x = y?=w429:bool)
        n219 = call "[ce] Boolean to Control Disable Status.vi"("Status in"=w429) -> ("Control Disable if True"=w428:u8)  [unwired: 3 in, 1 out]
        n220 = for {
          N: 11 -> [_]
          tunnel: w430 -> [w440]
          shift-right: [w438] -> w433
          shift-left: w432 -> [w437]
          shift-right: [w439] -> w434
          shift-left: w432 -> [w436]
          i -> [w441]
          n221 = Equal?(x=w441, y=w440) -> (x = y?=w442:bool)
          n222 = case shown="1" w441 {
            tunnel: w442 -> [w443 w449 _ w456 w461 w465 w469 w473 w475 w480 _]
            tunnel: w440 -> [_ _ _ _ _ _ _ _ _ _ w489]
            tunnel: [w444 w452 w453 w455 w459 w463 w467 w471 w476 w479 w485] -> w439
            tunnel: [w446 w450 w454 w457 w460 w464 w468 w472 w478 w482 w486] -> w438
            tunnel: w437 -> [w446 w451 w454 w458 w462 w466 w470 w474 w478 w482 w487]
            tunnel: w436 -> [w445 w452 w453 w455 w459 w463 w467 w471 w477 w481 w484]
            frame 0 {
              n223 = property on="str" class="Str"("Visible"=w443) -> ()  [unwired: 2 in, 2 out]
              n224 = property on="EnaWrap" class="Bool (strict)"("Visible"=w443) -> ()  [unwired: 2 in, 2 out]
              n225 = property on="h_str" class="Arr (strict)"("Visible"=w443) -> ()  [unwired: 2 in, 2 out]
              n226 = Or(x=w443, y=w445) -> (x .or. y?=w444:bool)
            }
            frame 1 {
              n227 = property on="dbl" class="DigNum (strict)"("Visible"=w449) -> ()  [unwired: 2 in, 2 out]
              n228 = property on="ShowInt32" class="Bool (strict)"("Visible"=w449) -> ("Value"=w448:bool)  [unwired: 2 in, 2 out]
              n229 = And(x=w449, y=w448) -> (x .and. y?=w447:bool)
              n230 = property on="h_dbl" class="Arr (strict)"("Visible"=w449) -> ()  [unwired: 2 in, 2 out]
              n231 = property on="I32M" class="DigNum (strict)"("Visible"=w447) -> ()  [unwired: 2 in, 2 out]
              n232 = property on="I32B" class="DigNum (strict)"("Visible"=w447) -> ()  [unwired: 2 in, 2 out]
              n233 = Or(x=w449, y=w451) -> (x .or. y?=w450:bool)
            }
            frame 2 {
            }
            frame 3 {
              n234 = property on="a1dbl" class="Arr (strict)"("Visible"=w456) -> ()  [unwired: 2 in, 2 out]
              n235 = property on="h_a1dbl" class="Arr (strict)"("Visible"=w456) -> ()  [unwired: 2 in, 2 out]
              n236 = Or(x=w456, y=w458) -> (x .or. y?=w457:bool)
            }
            frame 4 {
              n237 = property on="a2dbl" class="Arr (strict)"("Visible"=w461) -> ()  [unwired: 2 in, 2 out]
              n238 = property on="h_a2dbl" class="Arr (strict)"("Visible"=w461) -> ()  [unwired: 2 in, 2 out]
              n239 = Or(x=w461, y=w462) -> (x .or. y?=w460:bool)
            }
            frame 5 {
              n240 = property on="cdb" class="DigNum (strict)"("Visible"=w465) -> ()  [unwired: 2 in, 2 out]
              n241 = property on="h_cdb" class="Arr (strict)"("Visible"=w465) -> ()  [unwired: 2 in, 2 out]
              n242 = Or(x=w465, y=w466) -> (x .or. y?=w464:bool)
            }
            frame 6 {
              n243 = property on="a1cdb" class="Arr (strict)"("Visible"=w469) -> ()  [unwired: 2 in, 2 out]
              n244 = property on="h_a1cdb" class="Arr (strict)"("Visible"=w469) -> ()  [unwired: 2 in, 2 out]
              n245 = Or(x=w469, y=w470) -> (x .or. y?=w468:bool)
            }
            frame 7 {
              n246 = property on="a2cdb" class="Arr (strict)"("Visible"=w473) -> ()  [unwired: 2 in, 2 out]
              n247 = property on="h_a2cdb" class="Arr (strict)"("Visible"=w473) -> ()  [unwired: 2 in, 2 out]
              n248 = Or(x=w473, y=w474) -> (x .or. y?=w472:bool)
            }
            frame 8 {
              n249 = property on="a1str" class="Arr (strict)"("Visible"=w475) -> ()  [unwired: 2 in, 2 out]
              n250 = property on="h_a1str" class="Arr (strict)"("Visible"=w475) -> ()  [unwired: 2 in, 2 out]
              n251 = Or(x=w475, y=w477) -> (x .or. y?=w476:bool)
            }
            frame 9 {
              n252 = property on="a2str" class="Arr (strict)"("Visible"=w480) -> ()  [unwired: 2 in, 2 out]
              n253 = property on="h_a2str" class="Arr (strict)"("Visible"=w480) -> ()  [unwired: 2 in, 2 out]
              n254 = Or(x=w480, y=w481) -> (x .or. y?=w479:bool)
            }
            frame 10, Default {
              n255 = case shown="Default" w489 {
                tunnel: [FALSE TRUE FALSE] -> w483
                tunnel: [FALSE FALSE TRUE] -> w488
                tunnel: w487 -> [w491 w495 w499]
                tunnel: [w491 w495 w499] -> w486
                tunnel: [w490 w494 TRUE] -> w485
                tunnel: w484 -> [w490 w494 _]
                frame ..10 {
                }
                frame 252 {
                }
                frame Default {
                }
              }
              n256 = property on="any" class="Str"("Visible"=w488) -> ()  [unwired: 2 in, 2 out]
              n257 = property on="IR" class="Clust (strict)"("Visible"=w483) -> ()  [unwired: 2 in, 2 out]
              n258 = property on="h_any" class="Arr (strict)"("Visible"=w488) -> ()  [unwired: 2 in, 2 out]
              n259 = property on="h_IR" class="Arr (strict)"("Visible"=w483) -> ()  [unwired: 2 in, 2 out]
            }
          }
        }
        n260 = property on="%write" class="Bool"("DisabledEnum"=w428) -> ()  [unwired: 2 in, 2 out]
        n261 = property on="Precision" class="DigNum (strict)"("Visible"=w433) -> ()  [unwired: 2 in, 2 out]
        n262 = property on="Format" class="Ring (strict)"("Visible"=w433) -> ()  [unwired: 2 in, 2 out]
        n263 = property on="Display style" class="Ring (strict)"("Visible"=w434) -> ()  [unwired: 2 in, 2 out]
      }
      frame "EXIT" {
        n264 = Enqueue Element(queue=w504, element="EXIT") -> ()  [unwired: 2 in, 3 out]
        n265 = case shown="Default" w502 {
          frame "KeepFPOpen" {
          }
          frame Default {
            n266 = invoke class="VI" method="FP.Close"() -> ()  [unwired: 3 in, 3 out]
          }
        }
        n267 = Concatenate Strings("HALT;" ("string"), w507) -> (w506:string)
      }
      frame "HALT" {
        n268 = Release Queue(queue=w508) -> ()  [unwired: 2 in, 3 out]
      }
      frame "--------------------------------- 1" {
      }
      frame "Open FP" {
        n269 = invoke class="VI" method="FP.Open"("Activate"=TRUE ("Activate?"), "State"=T27."Standard") -> ()  [unwired: 3 in, 5 out]
      }
      frame "Set Window Size" {
        n270 = local read "%h_Show"() -> (w515:bool)
        n271 = property on="bndry" class="Str"() -> ("Bounds:Height"=w522:u32, "Position:Top"=w521:i32)  [unwired: 2 in, 2 out]
        n272 = property on="Context" class="Str"() -> ("Position:Top"=w523:i32)  [unwired: 2 in, 2 out]
        n273 = property class="VI"() -> (reference out=w532:refnum<vi>, "Front Panel Window:Panel Bounds"=w531:T30)  [unwired: 2 in, 1 out]
        n274 = Select(t="Resize Controls;", s=w515, f="") -> (s? t:f=w516:string)
        n275 = Compound Arithmetic op=ADD(w522, u32 0 ("Top"), w521) -> (w525:u32)
        n276 = Select(t=w525, s=w515, f=w521) -> (s? t:f=w524:u32)
        n277 = Unbundle By Name(w531) -> ("Top"=w529:i16)
        n278 = Subtract(x=w524, y=w523) -> (x-y=w527:u32)
        n279 = To Word Integer(number=w527) -> (16bit integer=w526:i16)
        n280 = Add(x=w529, y=w526) -> (x+y=w528:i16)
        n281 = Bundle By Name(cluster=w531, "Bottom"=w528) -> (w530:T30)
        n282 = property class="VI"(reference=w532, "Front Panel Window:Panel Bounds"=w530, "Front Panel.Resizeable"=w515) -> ()  [unwired: 1 in, 2 out]
        n283 = Concatenate Strings(w516, w533) -> (w519:string)
      }
      frame "Resize Controls" {
        n284 = case shown="252" w535 {
          tunnel: [_ w542 w543 w544 w545 w546 w547 w548 w549 w550 w551 w552] -> w534
          frame -1, 2 {
          }
          frame 0 {
            n285 = control-ref of="h_str"() -> (w542:refnum<vi>)
          }
          frame 1 {
            n286 = control-ref of="h_dbl"() -> (w543:refnum<vi>)
          }
          frame 3 {
            n287 = control-ref of="h_a1dbl"() -> (w544:refnum<vi>)
          }
          frame 4 {
            n288 = control-ref of="h_a2dbl"() -> (w545:refnum<vi>)
          }
          frame 5 {
            n289 = control-ref of="h_cdb"() -> (w546:refnum<vi>)
          }
          frame 6 {
            n290 = control-ref of="h_a1cdb"() -> (w547:refnum<vi>)
          }
          frame 7 {
            n291 = control-ref of="h_a2cdb"() -> (w548:refnum<vi>)
          }
          frame 8 {
            n292 = control-ref of="h_a1str"() -> (w549:refnum<vi>)
          }
          frame 9 {
            n293 = control-ref of="h_a2str"() -> (w550:refnum<vi>)
          }
          frame 10, Default {
            n294 = control-ref of="h_any"() -> (w551:refnum<vi>)
          }
          frame 252 {
            n295 = control-ref of="h_IR"() -> (w552:refnum<vi>)
          }
        }
        n296 = property on="Property Node" class="VI"() -> ("Front Panel.PanelBounds"=w539:T30)  [unwired: 2 in, 2 out]
        n297 = property on="Property Node" class="Arr"(reference=w534) -> (reference out=w537:refnum<vi>, error out=w538:errorcluster, "ClassName"=w536:string)  [unwired: 1 in]
        n298 = To Long Integer(number=w539) -> (32bit integer=w540:T31)
        n299 = case shown="\"String\"" w536 {
          tunnel: w537 -> [_ w572 w601]
          tunnel: w538 -> [_ w557 w592]
          tunnel: w540 -> [_ w554 w589]
          frame Default {
          }
          frame "String" {
            w571 = refnum<vi> refnum  # String
            n300 = To More Specific Class(target class=w571, reference=w572, error in=w557) -> (specific class reference=w556:refnum<vi>, error out=w555:errorcluster)
            n301 = property on="Property Node" class="Str"(reference=w556, error in=w555) -> (reference out=w569:refnum<vi>, error out=w570:errorcluster, "Position"=w568:T13)
            n302 = Unbundle(w554) -> ("Left"=w553:i32, "Top"=w565:i32, "Right"=w567:i32, "Bottom"=w566:i32)
            n303 = Unbundle(w568) -> ("Left"=w564:i32, "Top"=w563:i32)
            n304 = Compound Arithmetic op=ADD(w567, invert w553, invert w564, invert 3 ("value")) -> (w562:i32)
            n305 = Compound Arithmetic op=ADD(w566, invert w565, invert w563, invert 3 ("value")) -> (w561:i32)
            n306 = Bundle(w562, w561) -> (w560:cluster{i32, i32})  [unwired: 1 in]
            n307 = property on="Property Node" class="Str"(reference=w569, error in=w570, "Size"=w560) -> ()  [unwired: 2 out]
          }
          frame "Array" {
            w600 = refnum<vi> refnum  # Array
            n308 = To More Specific Class(target class=w600, reference=w601, error in=w592) -> (specific class reference=w591:refnum<vi>, error out=w590:errorcluster)
            n309 = Unbundle(w589) -> ("Left"=w588:i32, "Top"=w595:i32, "Right"=w597:i32, "Bottom"=w596:i32)
            n310 = property on="Property Node" class="Arr"(reference=w591, error in=w590) -> (reference out=w598:refnum<vi>, error out=w599:errorcluster, "Index Bnds"=w582:T30, "Array Element.Bounds"=w587:T12, "NumDims"=w574:u32)
            n311 = To Long Integer(number=w587) -> (32bit integer=w584:cluster{"Width":i32, "Height":i32})
            n312 = Unbundle(w582) -> ("Top"=w580:i16, "Right"=w581:i16)  [unwired: 2 out]
            n313 = Equal?(x=u32 2 ("y"), y=w574) -> (x = y?=w578:bool)
            n314 = Select(t=20 ("value"), s=w578, f=0) -> (s? t:f=w573:i32)
            n315 = Compound Arithmetic op=ADD(w597, invert w588, invert 5 ("value"), invert w581, invert w573) -> (w594:i32)
            n316 = Compound Arithmetic op=ADD(w596, invert w595, invert 5 ("value"), invert w580, invert w573) -> (w593:i32)
            n317 = Bundle(w594, w593) -> (w579:cluster{i32, i32})  [unwired: 1 in]
            n318 = Quotient & Remainder(x=w579, y=w584) -> (floor(x/y)=w583:cluster{i32, i32})  [unwired: 1 out]
            n319 = case shown="2" w574 {
              tunnel: w599 -> [_ w606 w611]
              tunnel: w598 -> [_ w605 w610]
              tunnel: w583 -> [_ w604 w609]
              frame 0, Default {
              }
              frame 1 {
                n320 = Unbundle(w604) -> (w603:i32)  [unwired: 1 out]
                n321 = property on="Property Node" class="Arr"(reference=w605, error in=w606, "Number of Columns"=u32 1, "Number of Rows"=w603) -> ()  [unwired: 2 out]
              }
              frame 2 {
                n322 = Unbundle(w609) -> (w608:i32, w607:i32)
                n323 = property on="Property Node" class="Arr"(reference=w610, error in=w611, "Number of Columns"=w608, "Number of Rows"=w607) -> ()  [unwired: 2 out]
              }
            }
          }
        }
      }
      frame "Control Appearance" {
        n324 = local read "%h_Show"() -> (w612:bool)
        n325 = call "[ce] Boolean to Control Disable Status.vi"("Status in"=w612) -> ("Control Disable if False"=w613:u8)  [unwired: 3 in, 1 out]
        n326 = property on="reversed order" class="Bool (strict)"("Disabled"=w613) -> ()  [unwired: 2 in, 2 out]
        n327 = property on="%h_Update" class="Bool"("Disabled"=w613) -> ()  [unwired: 2 in, 2 out]
        n328 = property on="%h_Auto" class="Bool (strict)"("Disabled"=w613) -> ()  [unwired: 2 in, 2 out]
      }
      frame "--------------------------------- 2" {
      }
      frame "Test Variable" {
        n329 = call "VM - Variable Info.vi"("VC Handle"=w627, "name_spec"=w626) -> ("error out"=w623:errorcluster, "alias"=w625:string, "has history"=w618:bool)  [unwired: 4 in, 3 out]
        n330 = feedback-in #2(w618) -> ()
        n331 = feedback #2() -> (w619:bool)  [unwired: 1 in]
        n332 = First Call?() -> (First Call?: T/F=w621:bool)
        n333 = Not Equal?(x=w618, y=w619) -> (x != y?=w620:bool)
        n334 = Or(x=w620, y=w621) -> (x .or. y?=w617:bool)
        n335 = case shown="No Error" w623 {
          tunnel: "alias" -> [w635 _]
          tunnel: w625 -> [w634 _]
          tunnel: w627 -> [w633 _]
          tunnel: w626 -> [w632 _]
          tunnel: w618 -> [w630 _]
          tunnel: w617 -> [w629 _]
          tunnel: [w628 "EXIT;"] -> w622
          tunnel: w616 -> [w628 _]
          frame No Error {
            n336 = case shown="True" w629 {
              tunnel: w630 -> [_ w637]
              frame False {
              }
              frame True {
                n337 = case shown="False" w637 {
                  selector: w637 -> [w638 _]
                  tunnel: [u8 2 ("Disabled") _] -> w636
                  frame False {
                    n338 = property on="%h_Show" class="Bool (strict)"("Val(Sgnl)"=w638) -> ()  [unwired: 2 in, 2 out]
                  }
                  frame True {
                  }
                }
                n339 = property on="show" class="Bool (strict)"("Disabled"=w636) -> ()  [unwired: 2 in, 2 out]
              }
            }
            n340 = Equal?(x=w635, y=w634) -> (x = y?=w631:bool)
            n341 = case shown="False" w631 {
              tunnel: w633 -> [w643 _]
              tunnel: w632 -> [w642 _]
              frame False {
                # "set new window title if\nalias name was changed"
                n342 = call "VM Spy - probe file name & win title.vi"("Variable"=w642, "VC Handle"=w643) -> ("alias"=w640:string, "probe win title"=w641:string)  [unwired: 3 in, 3 out]
                n343 = property class="VI"("Front Panel Window:Title"=w641) -> ()  [unwired: 2 in, 2 out]
                n344 = local write "alias"(w640) -> ()
              }
              frame True {
              }
            }
          }
          frame Error {
          }
        }
      }
      frame "Write Variable" {
        n345 = property on="Format" class="Ring (strict)"() -> ("Value"=w651:u8)  [unwired: 2 in, 2 out]
        n346 = property on="Precision" class="DigNum (strict)"() -> ("Value"=w650:u8)  [unwired: 2 in, 2 out]
        n347 = property on="ShowInt32" class="Bool (strict)"() -> ("Value"=w649:bool)  [unwired: 2 in, 2 out]
        n348 = property on="Display style" class="Ring (strict)"() -> ("Value"=w648:u32)  [unwired: 2 in, 2 out]
        n349 = property on="EnaWrap" class="Bool (strict)"() -> ("Value"=w647:bool)  [unwired: 2 in, 2 out]
        n350 = Bundle("Value"=w651, "Value"=w650, "Value"=w649, "Value"=w648, "Value"=w647) -> (w652:T32)  [unwired: 1 in]
        n351 = call "VM Spy - Dialog - Set Variable Value.vi"("Display params"=w652, "var name"=w645, "VC Handle"=w646) -> ()  [unwired: 8 in, 1 out]
      }
    }
  }
